vi "thermal_optical_capture_16.1.vi"() -> ()   [LabVIEW 2025]
uses:
  VIs_needed/Grab Manager Mode.ctl
  <vilib>/vision/driver/IMAQdx.llb/IMAQdx Buffer Number Mode.ctl
  <vilib>/vision/driver/NI_Vision_Acquisition_Software.lvlib
  <resource>/objmgr/imaqdx.rc
panel:
  in  "milliseconds to wait":u32=100
  out "Optical Frame Out":string
  in  "Stop":bool
  out "Images Saved Per Second":dbl
  out "Images Behind":i32
  out "Images Acquired Per Second":dbl
  in  "Skip Count":u32
  out "Write Speed Waveform":dbl(graph) caption="Image File Write Speed"
  in  "Number of Images":u32=30
  in  "Camera Name":refnum<k21> caption="IMAQdx Session"
  out "Thermal Preview":T1(plugin-control)
  in  "Stop Preview":bool
  out "Time  b/w Frames":u32
  in  "STOP ACQUISITION":bool
  in  "Focus":dbl(slide) scale=0.0..100.0
  out "Thermal Frame Out":string
  in  "Output Folder":path
  in  "thermal capture interval (s)":dbl
  in  "Flag Button":bool
  in  "Stop & Save":bool
  in  "Record":bool
  # "Instructions:\n1) Make sure terminal is closed (from previous sessions)\n2) Input data folder path and milliseconds to wait (~100)\n3) Run VI. (Optical images will begin writing, disregard.)\n4) Wait until terminal gives \"thermal camera calibrated and data reliable\" message\n5) Press Thermal Record \"Start\", both thermal & optical will write files with common timestamps"
  # "Thermal Record"
  # "(Enter \"28\")"
  # "^ append to base data folder \"...\\raw\\test_n\" for nth recording"
  # "(applies to thermal)"
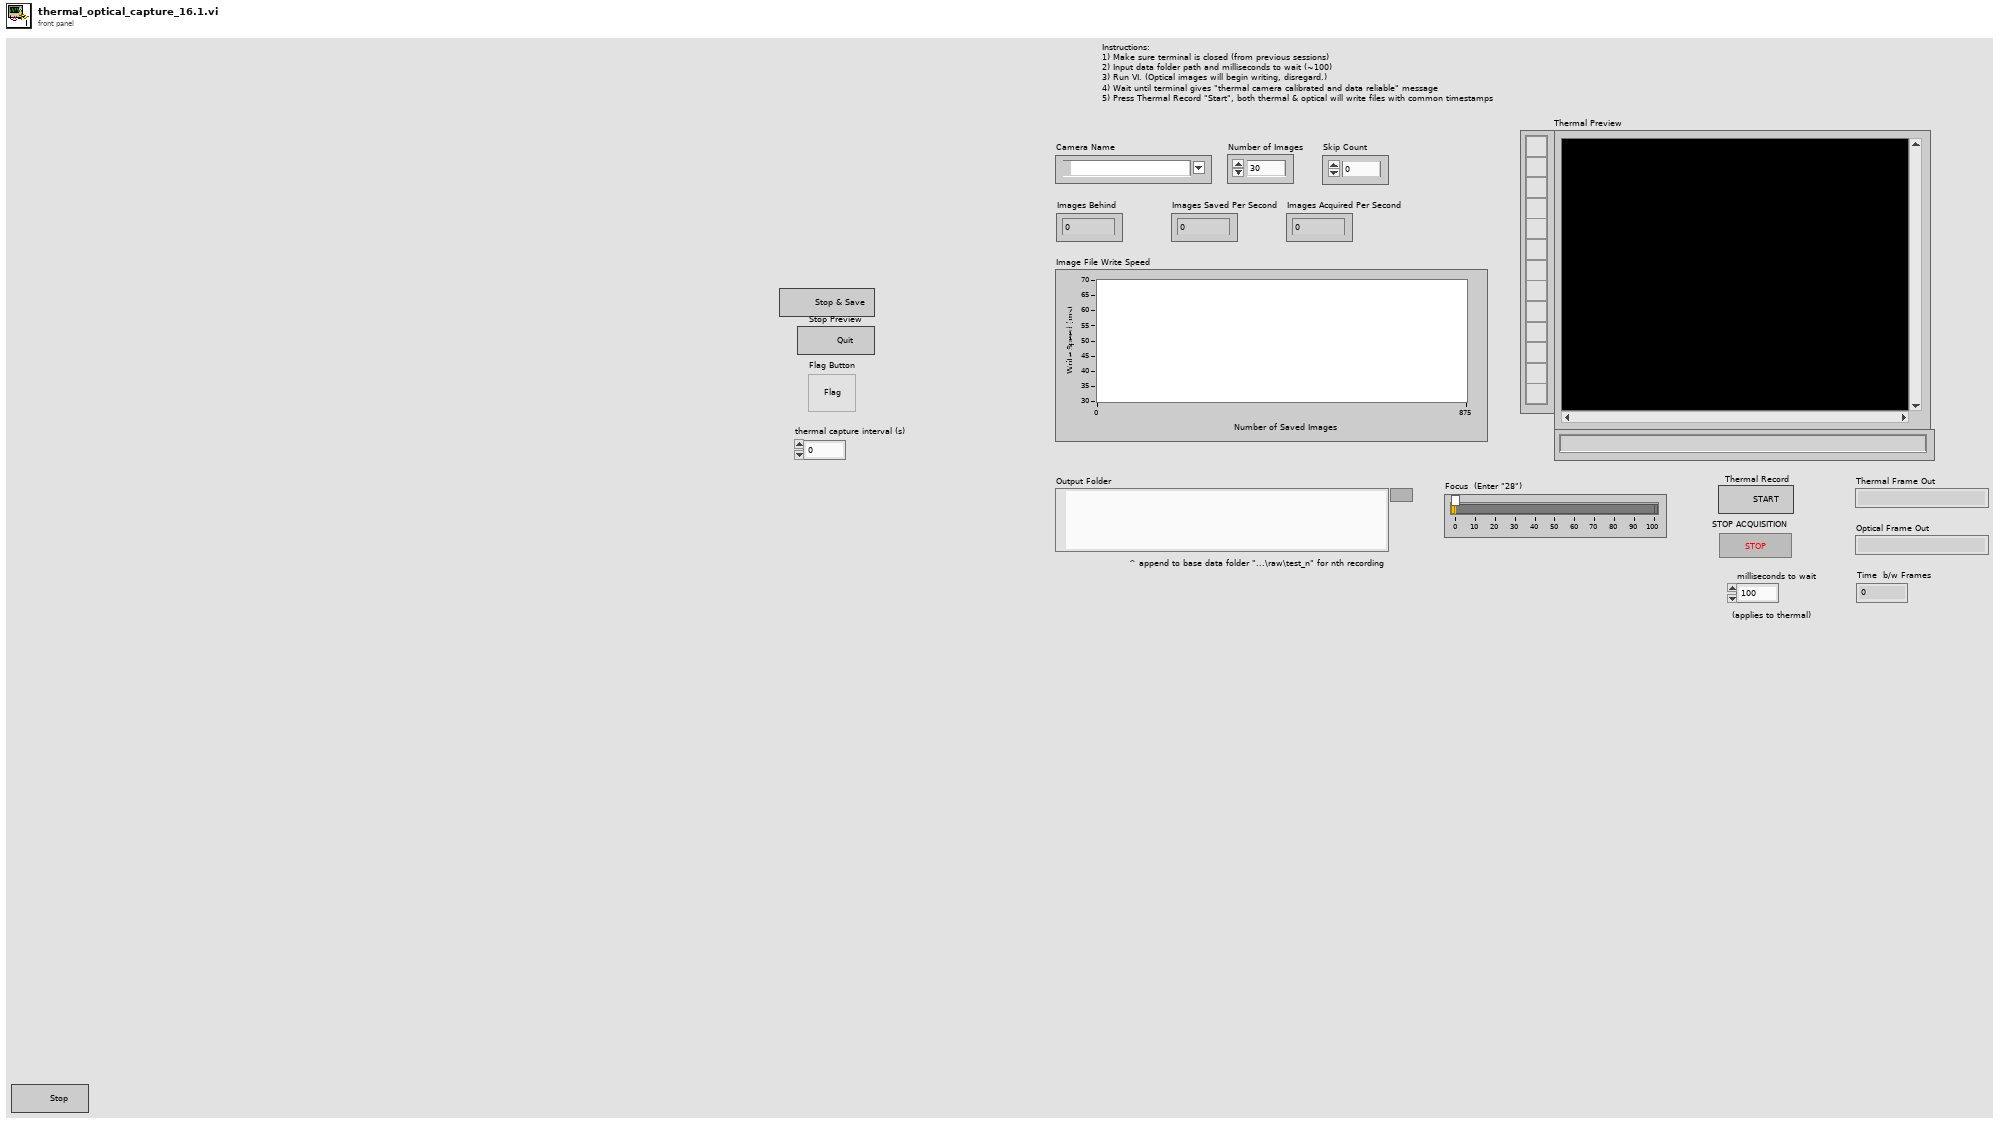
[diagram p1: front panel]
types:
  T1 = typedef "IMAQ Image.ctl" = refnum<image>
  T2 = typedef "Grab Manager Mode.ctl" = enum16{"Create Processing Images", "Lock", "Add Acquired Image", "Get Acquired Image", "Unlock", "Dispose Processing Images"}
  T3 = cluster{"Number of Processing Images":u32, "Image Border Size":u32}
  T4 = enum16{"open", "replace", "create", "open or create", "replace or create", "replace or create with confirmation"}
  T5 = enum16{"big-endian, network order", "native, host order", "little-endian"}
  T6 = typedef "NI_Vision_Acquisition_Software.lvlib/IMAQdx Buffer Number Mode.ctl" = enum32{"Next", "Last", "Buffer Number", "Every", "Last New"}
  T7 = typedef "Image Type" = u32
  T8 = typedef "IMAQdx.ctl" = refnum<k21>
  T9 = enum16{"Standard", "Buffered", "CRLF", "Immediate"}
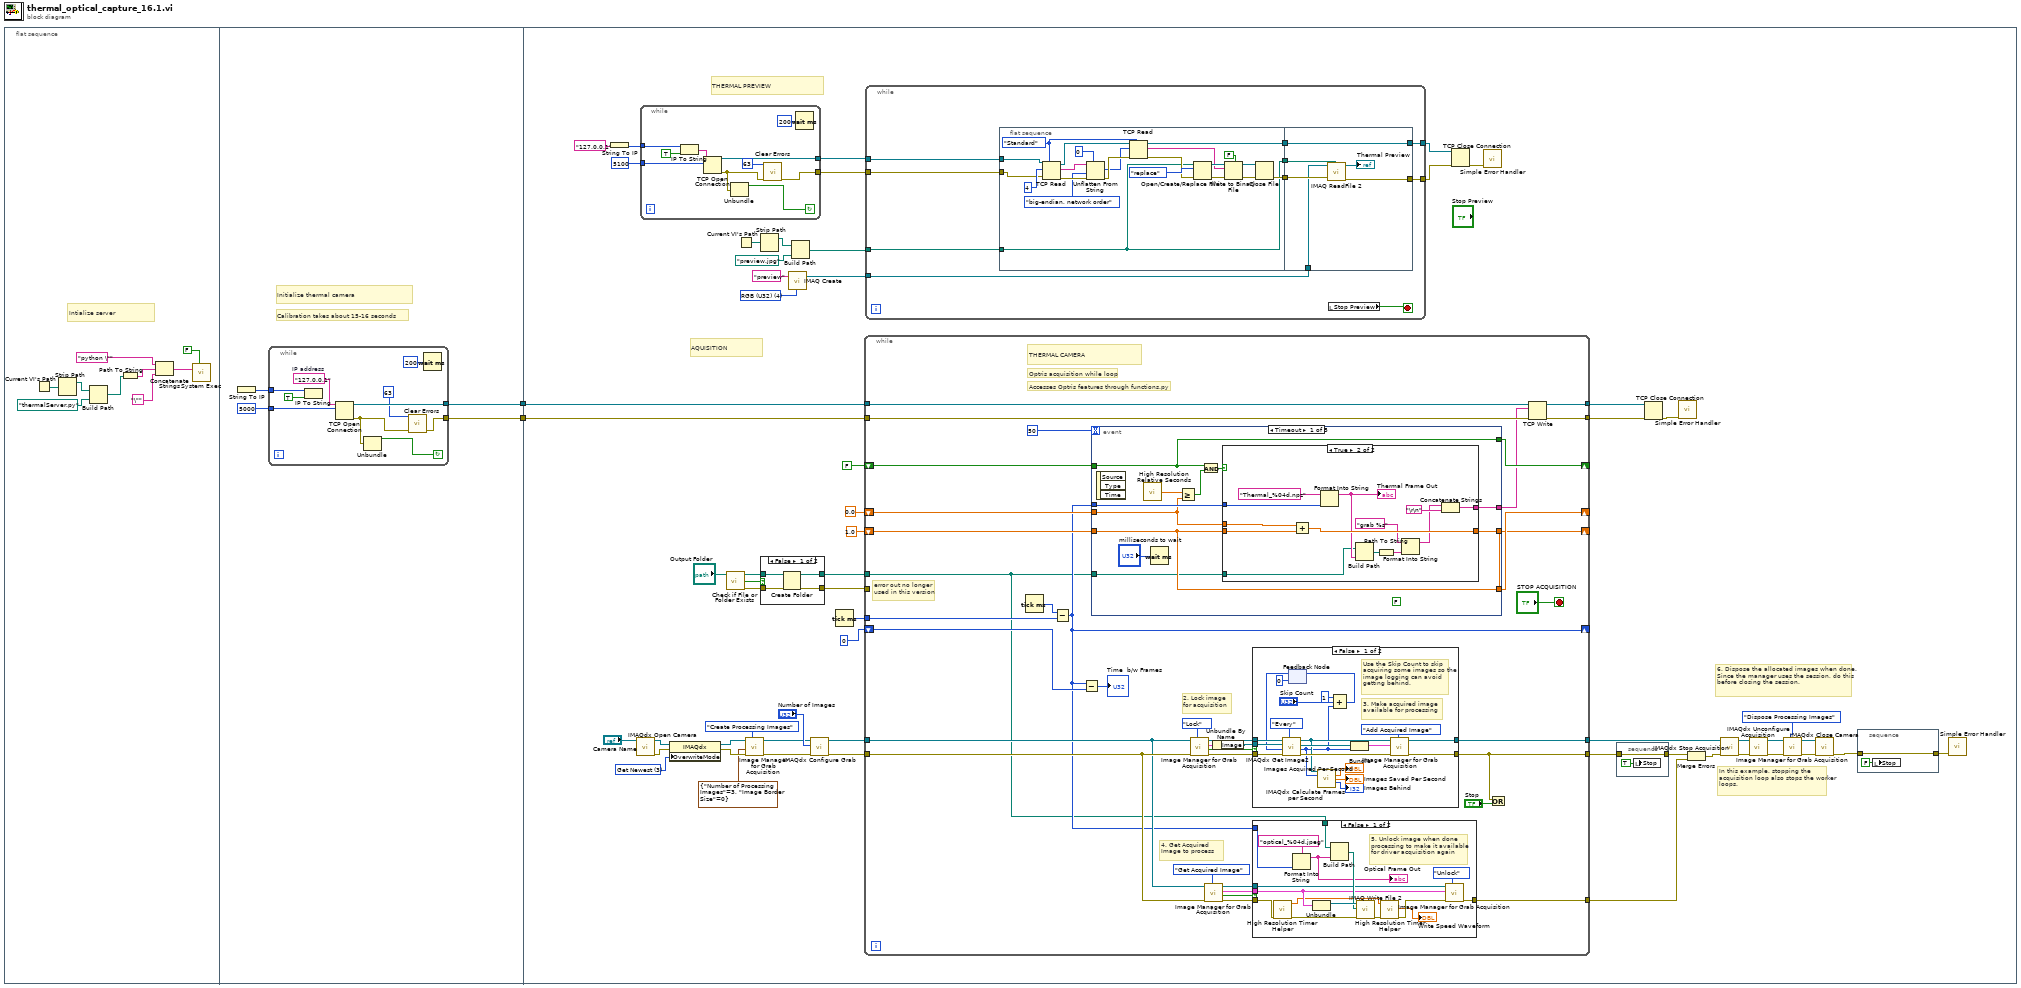
[diagram p0: block diagram]
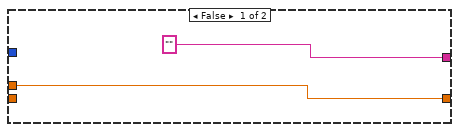
[diagram p5: hidden frame]
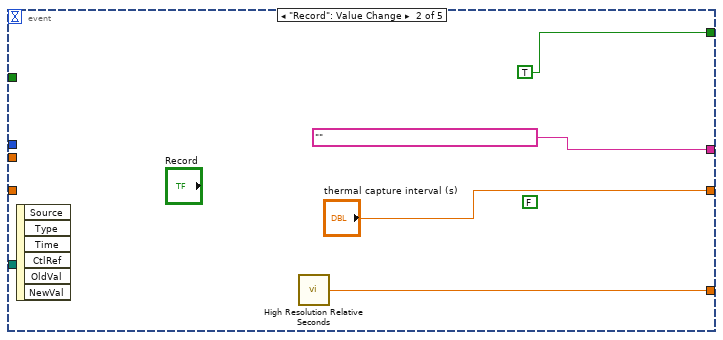
[diagram p6: hidden frame]
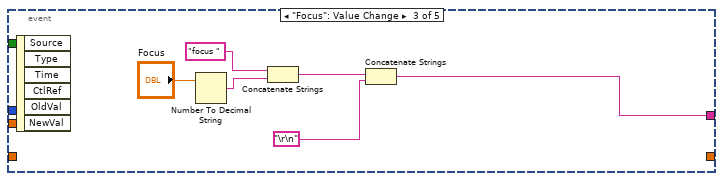
[diagram p7: hidden frame]
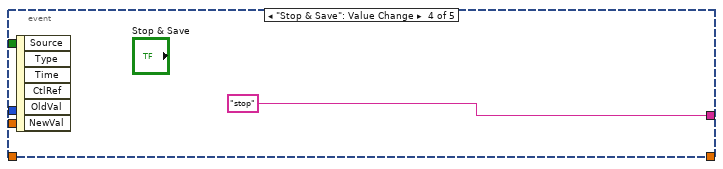
[diagram p8: hidden frame]
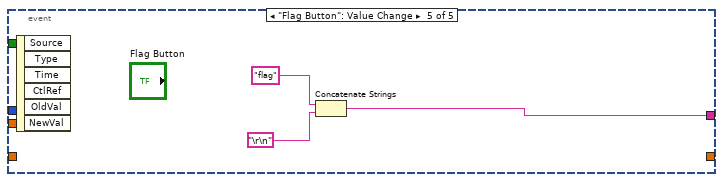
[diagram p9: hidden frame]
diagram:
  n1 = flat-sequence {
    tunnel: [w13] -> w2
    tunnel: [w12] -> w1
    tunnel: w1 -> [w79]
    tunnel: w2 -> [w78]
    frame #0 {
      # "Intialize server"
      n2 = Current VI's Path() -> (path=w6:path)
      n3 = Strip Path(path=w6) -> (stripped path=w7:path)  [unwired: 1 out]
      n4 = Build Path(base path=w7, name or relative path=path "thermalServer.py") -> (appended path=w4:path)
      n5 = Path To String(path=w4) -> (string=w10:string)
      n6 = Concatenate Strings("python \"" ("string"), w10, "\"" ("string")) -> (w9:string)
      n7 = call <vilib>:"System Exec.vi"("wait until completion? (T)"=FALSE, "command line"=w9) -> ()  [unwired: 6 in, 4 out]
    }
    frame #1 {
      # "Initialize thermal camera"
      # "Calibration takes about 15-16 seconds"
      n8 = String To IP() -> (0:w15:u32)  [unwired: 1 in]
      n9 = while {
        tunnel: [w20] -> w13
        tunnel: [w25] -> w12
        tunnel: w15 -> [w24]
        tunnel: u16 5000 ("remote port or service name") -> [w22]
        stop <- w17 continue-if-true
        w16 = "127.0.0.1"  # IP address
        n10 = IP To String(1:TRUE ("dot notation? (F)"), 2:w24) -> ()  [unwired: 1 out]
        n11 = TCP Open Connection(address=w16, remote port or service name=w22) -> (connection ID=w25:refnum<k5>, error out=w21:errorcluster)  [unwired: 3 in]
        n12 = Unbundle(w21) -> ("status"=w17:bool)  [unwired: 2 out]
        n13 = call <vilib>:"Clear Errors.vi"("error in (no error)"=w21, "specific error code to clear (0: all)"=63) -> ("error out"=w20:errorcluster)  [unwired: 4 in, 1 out]
        n14 = Wait (ms)(milliseconds to wait=u32 200) -> ()  [unwired: 1 out]
      }
    }
    frame #2 {
      w33 = u32 3 items=["Get Oldest"=0, "Fail"=2, "Get Newest"=3] ("OverwriteMode")
      w66 = T7 4 items=["Grayscale (U8)", "Grayscale (I16)", "Grayscale (SGL)", "Complex (CSG)", "RGB (U32)", "HSL (U32)", "RGB (U64)", "Grayscale (U16)"] ("Image Type")
      # "6. Dispose the allocated images when done. Since the manager uses the session, do this before closing the session."
      # "In this example, stopping the acquisition loop also stops the worker loops."
      # "THERMAL PREVIEW"
      # "AQUISITION"
      n15 = String To IP(1:"127.0.0.1" ("name")) -> (0:w65:u32)
      n16 = call <vilib>:"IMAQdx Open Camera.vi"("Session In"="Camera Name") -> ("error out"=w48:errorcluster, "Session Out"=w49:T8)  [unwired: 2 in, 7 out]
      n17 = while {
        tunnel: w65 -> [w102]
        tunnel: [w96] -> w64
        tunnel: [w100] -> w63
        tunnel: u16 5100 ("remote port or service name") -> [w98]
        stop <- w93 continue-if-true
        n18 = IP To String(1:TRUE ("dot notation? (F)"), 2:w102) -> (0:w101:string)
        n19 = TCP Open Connection(address=w101, remote port or service name=w98) -> (connection ID=w100:refnum<k5>, error out=w97:errorcluster)  [unwired: 3 in]
        n20 = Unbundle(w97) -> ("status"=w93:bool)  [unwired: 2 out]
        n21 = call <vilib>:"Clear Errors.vi"("error in (no error)"=w97, "specific error code to clear (0: all)"=63) -> ("error out"=w96:errorcluster)  [unwired: 4 in, 1 out]
        n22 = Wait (ms)(milliseconds to wait=u32 200) -> ()  [unwired: 1 out]
      }
      n23 = property class="IMAQdx"(reference=w49, error in=w48, "OverwriteMode"=w33) -> (reference out=w51:T8, error out=w50:errorcluster)
      n24 = call <vilib>:"Check if File or Folder Exists.vi"("path"="Output Folder") -> ("error out"=w58:errorcluster, "file or folder exists?"=w60:bool)  [unwired: 8 in, 1 out]
      n25 = Current VI's Path() -> (path=w71:path)
      n26 = call "Image Manager for Grab Acquisition.vi"("Mode"=Grab_Manager_Mode."Create Processing Images", "error in (no error)"=w50, "Init Settings"=T3 {"Number of Processing Images"=3, "Image Border Size"=0}, "Session In"=w51) -> ("error out"=w46:errorcluster, "Session Out"=w45:T8)  [unwired: 4 in, 2 out]
      n27 = Strip Path(path=w71) -> (stripped path=w72:path)  [unwired: 1 out]
      n28 = case shown="False" w60 {
        tunnel: "Output Folder" -> [w90 w92]
        tunnel: [w89 w92] -> w53
        tunnel: w58 -> [w88 w91]
        tunnel: [w87 w91] -> w57
        frame False {
          n29 = Create Folder(path (use dialog)=w90, error in=w88) -> (created path=w89:path, error out=w87:errorcluster)  [unwired: 1 in, 1 out]
        }
        frame True {
        }
      }
      n30 = call "IMAQ Create"("Image Name"="preview", "Image Type"=w66) -> ("New Image"=w69:T1)  [unwired: 3 in, 1 out]
      n31 = Build Path(base path=w72, name or relative path=path "preview.jpg") -> (appended path=w70:path)
      n32 = call <vilib>:"IMAQdx Configure Grab.vi"("error in"=w46, "Number of Buffers"="Number of Images", "Session In"=w45) -> ("error out"=w30:errorcluster, "Session Out"=w29:T8)  [unwired: 7 in]
      n33 = Tick Count (ms)() -> (millisecond timer value=w74:u32)
      n34 = while {
        tunnel: [w176] -> w80
        tunnel: [w175] -> w81
        tunnel: w79 -> [w174]
        tunnel: w78 -> [w173]
        shift-right: [w172] -> _
        shift-left: 0.0 -> [w169]
        shift-right: [w170] -> _
        shift-left: 1.0 -> [w167]
        shift-right: [w171] -> _
        shift-left: FALSE -> [w168]
        tunnel: w74 -> [w166]
        shift-right: [w142] -> _
        shift-left: u32 0 -> [w165]
        tunnel: w53 -> [w141]
        tunnel: w57 -> [_]
        tunnel: w30 -> [w147]
        tunnel: w29 -> [w146]
        tunnel: [w145] -> w28
        tunnel: [w144] -> w27
        tunnel: [w143] -> w26
        stop <- "STOP ACQUISITION" stop-if-true
        # "4. Get Acquired Image to process"
        # "2. Lock image for acquisition"
        # "error out no longer used in this version"
        # "THERMAL CAMERA"
        # "Optris acquisition while loop"
        # "Accesses Optris features through functions.py"
        n35 = Tick Count (ms)() -> (millisecond timer value=w161:u32)
        n36 = Subtract(x=w161, y=w166) -> (x-y=w142:u32)
        n37 = Subtract(x=w142, y=w165) -> (x-y=→"Time  b/w Frames":u32)
        n38 = event shown="[0] Timeout" {
          selector: _ -> [_ _ _ _ _]
          dyn-events: _ -> [_ _ _ _ _]
          timeout: 50 -> [_ _ _ _ _]
          tunnel: [w222 "" w246 "stop" w255] -> w162
          tunnel: w142 -> [w223 _ _ _ _]
          tunnel: [w220 w245 _ _ _] -> w172
          tunnel: [w218 TRUE _ _ _] -> w171
          tunnel: [w219 "thermal capture interval (s)" _ _ _] -> w170
          tunnel: w169 -> [w221 _ _ _ _]
          tunnel: w168 -> [w218 _ _ _ _]
          tunnel: w167 -> [w219 _ _ _ _]
          tunnel: w141 -> [w217 _ _ _ _]
          event Timeout {
            (unwired) FALSE
            n39 = event-data() -> ()  [unwired: 1 in, 3 out]
            n40 = call <vilib>:"High Resolution Relative Seconds.vi"() -> ("relative seconds"=w226:dbl)
            n41 = Wait (ms)(milliseconds to wait="milliseconds to wait") -> ()  [unwired: 1 out]
            n42 = Greater Or Equal?(x=w226, y=w221) -> (x >= y?=w225:bool)
            n43 = And(x=w218, y=w225) -> (x .and. y?=w224:bool)
            n44 = case shown="True" w224 {
              tunnel: w223 -> [_ w239]
              tunnel: ["" w240] -> w222
              tunnel: w221 -> [w227 w238]
              tunnel: w219 -> [_ w237]
              tunnel: [w227 w236] -> w220
              tunnel: w217 -> [_ w229]
              frame False {
              }
              frame True {
                n45 = Add(x=w238, y=w237) -> (x+y=w236:dbl)
                n46 = Format Into String(format string="Thermal_%04d.npz", w239) -> (resulting string=w230:string)  [unwired: 2 in, 1 out]
                "Thermal Frame Out" <- w230
                n47 = Build Path(base path=w229, name or relative path=w230) -> (appended path=w234:path)
                n48 = Path To String(path=w234) -> (string=w232:string)
                n49 = Format Into String(format string="grab %s", w232) -> (resulting string=w231:string)  [unwired: 2 in, 1 out]
                n50 = Concatenate Strings(w231, "\r\n") -> (w240:string)
              }
            }
          }
          event "Record": Value Change {
            (unwired) FALSE
            n51 = event-data() -> ()  [unwired: 1 in, 6 out]
            n52 = call <vilib>:"High Resolution Relative Seconds.vi"() -> ("relative seconds"=w245:dbl)
          }
          event "Focus": Value Change {
            n53 = event-data() -> ()  [unwired: 1 in, 6 out]
            n54 = Number To Decimal String(number="Focus") -> (decimal integer string=w251:string)  [unwired: 1 in]
            n55 = Concatenate Strings("focus ", w251) -> (w248:string)
            n56 = Concatenate Strings(w248, "\r\n") -> (w246:string)
          }
          event "Stop & Save": Value Change {
            n57 = event-data() -> ()  [unwired: 1 in, 6 out]
          }
          event "Flag Button": Value Change {
            n58 = event-data() -> ()  [unwired: 1 in, 6 out]
            n59 = Concatenate Strings("flag", "\r\n") -> (w255:string)
          }
        }
        n60 = call "Image Manager for Grab Acquisition.vi"("Mode"=Grab_Manager_Mode."Lock", "error in (no error)"=w147, "Session In"=w146) -> ("error out"=w153:errorcluster, "No Available Image"=w152:bool, "Image Settings Out"=w154:cluster{"Image":T1, "Buffer Number":u32}, "Session Out"=w151:T8)  [unwired: 5 in]
        n61 = call "Image Manager for Grab Acquisition.vi"("Mode"=Grab_Manager_Mode."Get Acquired Image", "error in (no error)"=w147, "Session In"=w146) -> ("error out"=w158:errorcluster, "No Available Image"=w156:bool, "Image Settings Out"=w157:cluster{"Image":T1, "Buffer Number":u32}, "Session Out"=w159:T8)  [unwired: 5 in]
        n62 = Unbundle By Name(w154) -> ("Image"=w155:T1)
        n63 = case shown="False" w152 {
          tunnel: [w205 w215] -> w144
          tunnel: [w204 w214] -> w143
          tunnel: w151 -> [w213 w215]
          tunnel: w153 -> [w212 w214]
          tunnel: w155 -> [w206 _]
          frame False {
            # "3. Make acquired image available for processing"
            # "Use the Skip Count to skip acquiring some images so the image logging can avoid getting behind."
            n64 = feedback #1(u32 0) -> (w195:u32)
            n65 = call <vilib>:"IMAQdx Get Image2.vi"("Buffer Number Mode (Next)"=IMAQdx_Buffer_Number_Mode."Every", "error in"=w212, "Buffer Number In"=w195, "Image In"=w206, "Session In"=w213) -> ("error out"=w208:errorcluster, "Buffer Number Out"=w199:u32, "Image Out"=w210:T1, "Session Out"=w203:T8)  [unwired: 3 in]
            n66 = call <vilib>:"IMAQdx Calculate Frames per Second.vi"("Session In"=w203, "Buffer Number"=w199) -> ("Acquired Frames per Second"=→"Images Acquired Per Second":dbl, "Processed Frames per Second"=→"Images Saved Per Second":dbl, "Images Behind"=→"Images Behind":i32)  [unwired: 7 in, 4 out]
            n67 = Compound Arithmetic op=ADD(u32 1 ("value"), "Skip Count", w199) -> (w196:u32)
            n68 = feedback-in #1(w196) -> ()
            n69 = Bundle("Image Out"=w210, "Buffer Number Out"=w199) -> (w209:cluster{"Image Out":T1, "Buffer Number Out":u32})  [unwired: 1 in]
            n70 = call "Image Manager for Grab Acquisition.vi"("Mode"=Grab_Manager_Mode."Add Acquired Image", "error in (no error)"=w208, "Image Settings In"=w209, "Session In"=w203) -> ("error out"=w204:errorcluster, "Session Out"=w205:T8)  [unwired: 4 in, 2 out]
          }
          frame True {
            # "The Lock function already has a delay inside when no images are available to prevent loop from going too fast and starving the worker threads from getting processing time."
            # "Write to disk operation is taking longer so images aren't added back to manager. Wait until there is an available image"
          }
        }
        n71 = case shown="False" w156 {
          tunnel: w158 -> [w185 w193]
          tunnel: w157 -> [w187 _]
          tunnel: [w189 w193] -> w145
          tunnel: w159 -> [w186 _]
          tunnel: w142 -> [w179 _]
          tunnel: w141 -> [w178 _]
          frame False {
            # "5. Unlock image when done processing to make it available for driver acquisition again"
            n72 = call "High Resolution Timer Helper.vi"("error in (no error)"=w185) -> ("error out"=w184:errorcluster, "Current Time"=w180:dbl)  [unwired: 8 in, 1 out]
            n73 = Format Into String(format string="optical_%04d.jpeg", w179) -> (resulting string=w177:string)  [unwired: 2 in, 1 out]
            "Optical Frame Out" <- w177
            n74 = Unbundle(w187) -> ("Image"=w192:T1)  [unwired: 1 out]
            n75 = Build Path(base path=w178, name or relative path=w177) -> (appended path=w190:path)
            n76 = call-poly "IMAQ Write File 2"("error in (no error)"=w184, "File Path"=w190, "Image"=w192) -> ("error out"=w183:errorcluster)  [unwired: 7 in, 1 out]
            n77 = call "High Resolution Timer Helper.vi"("error in (no error)"=w183, "Previous Time"=w180) -> ("error out"=w182:errorcluster, "Time Difference (ms)"=→"Write Speed Waveform":dbl)  [unwired: 7 in, 1 out]
            n78 = call "Image Manager for Grab Acquisition.vi"("Mode"=Grab_Manager_Mode."Unlock", "error in (no error)"=w182, "Image Settings In"=w187, "Session In"=w186) -> ("error out"=w189:errorcluster)  [unwired: 4 in, 3 out]
          }
          frame True {
            # "No acquired images to process"
          }
        }
        n79 = Or(x=w143, y="Stop") -> ()  [unwired: 1 out]
        n80 = TCP Write(connection ID=w174, data in=w162, error in (no error)=w173) -> (connection ID out=w175:refnum<k5>, error out=w176:errorcluster)  [unwired: 1 in, 1 out]
      }
      n81 = while {
        tunnel: w69 -> [w107]
        tunnel: [w108] -> w55
        tunnel: [w112] -> w54
        tunnel: w70 -> [w110]
        tunnel: w64 -> [w105]
        tunnel: w63 -> [w104]
        stop <- w103 stop-if-true
        n82 = flat-sequence {
          tunnel: w110 -> [w116]
          tunnel: [w118] -> w111
          tunnel: [w117] -> w109
          tunnel: [w116] -> w106
          tunnel: w105 -> [w114]
          tunnel: w104 -> [w113]
          tunnel: [w140] -> w112
          tunnel: w111 -> [w140]
          tunnel: w109 -> [w139]
          tunnel: [w138] -> w108
          tunnel: w107 -> [w137]
          tunnel: w106 -> [w136]
          frame #0 {
            w127 = T9."Standard" ("mode (standard)")
            n83 = TCP Read(connection ID=w113, bytes to read=4, error in (no error)=w114, 7:w127) -> (connection ID out=w130:refnum<k5>, data out=w115:string, error out=w133:errorcluster)  [unwired: 1 in]
            n84 = Unflatten From String(type=0, binary string=w115, byte order (0:big-endian, network order)=T5."big-endian, network order", error in (no error)=w133) -> (value=w128:i32, error out=w129:errorcluster)  [unwired: 1 in, 1 out]
            n85 = TCP Read(connection ID=w130, bytes to read=w128, error in (no error)=w129, 7:w127) -> (connection ID out=w118:refnum<k5>, data out=w123:string, error out=w125:errorcluster)  [unwired: 1 in]
            n86 = Open/Create/Replace File(file path (use dialog)=w116, error in=w125, operation (0:open)=T4."replace") -> (refnum out=w124:refnum<file>, error out=w121:errorcluster)  [unwired: 3 in, 1 out]
            n87 = Write to Binary File(file (use dialog)=w124, data=w123, error in=w121, 5:FALSE ("prepend array or string size? (T)")) -> (refnum out=w119:refnum<file>, error out=w120:errorcluster)  [unwired: 2 in, 1 out]
            n88 = Close File(refnum=w119, error in=w120) -> (error out=w117:errorcluster)  [unwired: 1 out]
          }
          frame #1 {
            n89 = call "IMAQ ReadFile 2"("File Path"=w136, "error in (no error)"=w139, "Image"=w137) -> ("error out"=w138:errorcluster, "Image Out"=→"Thermal Preview":T1)  [unwired: 4 in, 3 out]
          }
        }
        n90 = local read "Stop Preview"() -> (w103:bool)
      }
      n91 = TCP Close Connection(connection ID=w54, error in (no error)=w55) -> (error out=w56:errorcluster)  [unwired: 1 in, 1 out]
      n92 = call <vilib>:"Simple Error Handler.vi"("error in (no error)"=w56) -> ()  [unwired: 4 in, 5 out]
      n93 = stacked-sequence {
        tunnel: [w85] -> w41
        tunnel: w26 -> [w85]
        frame #0 {
          n94 = local write "Stop"(TRUE ("Stop")) -> ()
        }
      }
      n95 = TCP Close Connection(connection ID=w81, error in (no error)=w80) -> (error out=w82:errorcluster)  [unwired: 1 in, 1 out]
      n96 = call <vilib>:"Simple Error Handler.vi"("error in (no error)"=w82) -> ()  [unwired: 4 in, 5 out]
      n97 = Merge Errors(w41, w28) -> (w42:errorcluster)
      n98 = call <vilib>:"IMAQdx Stop Acquisition.vi"("error in"=w42, "Session In"=w27) -> ("error out"=w43:errorcluster, "Session Out"=w44:T8)  [unwired: 8 out]
      n99 = call <vilib>:"IMAQdx Unconfigure Acquisition.vi"("error in"=w43, "Session In"=w44) -> ("error out"=w38:errorcluster, "Session Out"=w39:T8)  [unwired: 8 out]
      n100 = call "Image Manager for Grab Acquisition.vi"("Mode"=Grab_Manager_Mode."Dispose Processing Images", "error in (no error)"=w38, "Session In"=w39) -> ("error out"=w36:errorcluster, "Session Out"=w37:T8)  [unwired: 5 in, 2 out]
      n101 = call <vilib>:"IMAQdx Close Camera.vi"("error in"=w36, "Session In"=w37) -> ("error out"=w35:errorcluster)  [unwired: 9 out]
      n102 = stacked-sequence {
        tunnel: [w83] -> w40
        tunnel: w35 -> [w83]
        frame #0 {
          n103 = local write "Stop"(FALSE ("Stop")) -> ()
        }
      }
      n104 = call <vilib>:"Simple Error Handler.vi"("error in (no error)"=w40) -> ()  [unwired: 4 in, 5 out]
    }
  }
